vi "ZM-PC-EP-create.vi"(8 "error in (no error)":errorcluster, 10 "error_to_report":errorcluster, 11 "sender":string) -> (0 "error out":errorcluster, 3 "package":refnum<class "ZM-PC-EP-error_package.lvclass">)   [LabVIEW 2020, in "ZM-PC-packages.lvlib" / "ZM-PC-EP-error_package.lvclass"]
doc: "Creates an error package addressed to Root: initialises it and writes sender, code and source as its data (error_to_report is data here, not the error chain). Returns it as a ZM-PC-EP-error_package."
uses:
  ZM-PC-EP-error_package.lvclass
  ZM-PC-EP-error_package.lvclass/ZM-PC-EP-error_package.ctl
  ZM-PC-package/ZM-PC-package.lvclass
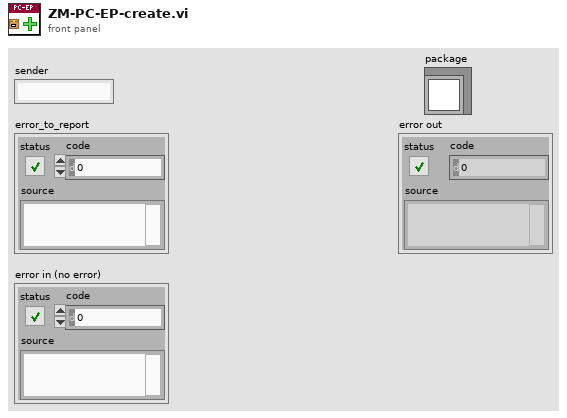
[diagram p1: front panel]
types:
  T1 = enum16{"Unknown", "Root", "Hardware", "Communication"}
  T2 = cluster{"sender":string, "code":i32, "source":string}
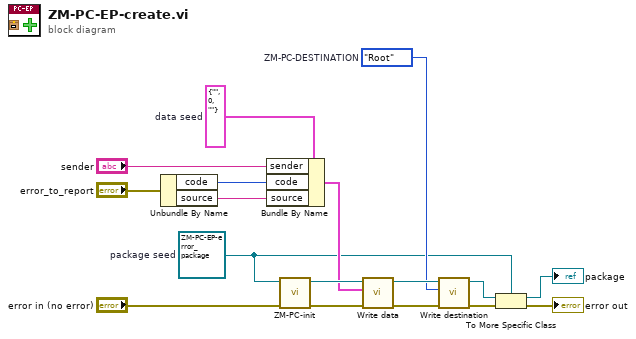
[diagram p0: block diagram]
diagram:
  w6 = T1."Root"  # ZM-PC-DESTINATION
  w12 = T2 {"sender"="", "code"=0, "source"=""}  # data seed
  w3 = refnum<class "ZM-PC-EP-error_package.lvclass"> refnum  # package seed
  n1 = Unbundle By Name("error_to_report") -> ("code"=w14:i32, "source"=w13:string)
  n2 = Bundle By Name(cluster=w12, "sender"="sender", "code"=w14, "source"=w13) -> (w9:T2)
  n3 = call-dynamic "ZM-PC-init.vi"("error in (no error)"="error in (no error)", "ZM-PC-EP-error_package in"=w3) -> ("error out"=w11:errorcluster, "ZM-PC-EP-error_package out"=w10:refnum<class "ZM-PC-EP-error_package.lvclass">)  [unwired: 8 in]
  n4 = call "Write data.vi"("error in (no error)"=w11, "ZM-PC-EP-DATA"=w9, "ZM-PC-EP-error_package in"=w10) -> ("error out"=w8:errorcluster, "ZM-PC-EP-error_package out"=w7:refnum<class "ZM-PC-EP-error_package.lvclass">)  [unwired: 7 in]
  n5 = call "Write destination.vi"("error in (no error)"=w8, "ZM-PC-DESTINATION"=w6, "ZM-PC-package in"=w7) -> ("error out"=w4:errorcluster, "ZM-PC-package out"=w5:refnum<class "ZM-PC-EP-error_package.lvclass">)  [unwired: 7 in]
  n6 = To More Specific Class(target class=w3, reference=w5, error in=w4) -> (specific class reference=→"package":refnum<class "ZM-PC-EP-error_package.lvclass">, error out=→"error out":errorcluster)
